vi "Check interlock status.vi"(8 "error in":errorcluster, 11 "VISA resource name":refnum<visa-resource-name>) -> (0 "error out":errorcluster, 3 "Boolean":bool)   [LabVIEW 2021]
uses:
  HI-POT_Driver/GPT-9800_GSB_L8.5/GPT-9000.lvlib
panel:
  out "Query the function test status":string
  out "Return  the test status":string
  out "RESULT":bool
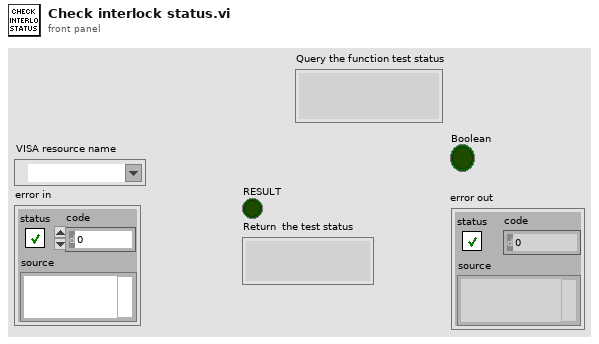
[diagram p1: front panel]
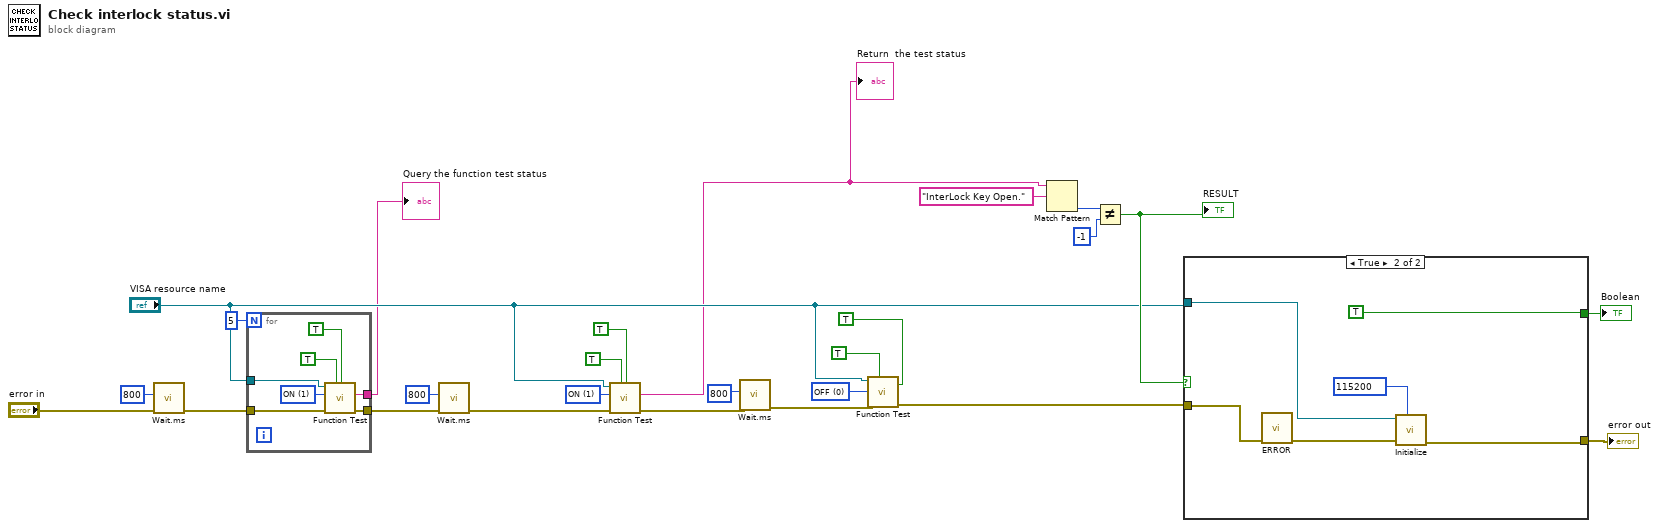
[diagram p0: block diagram]
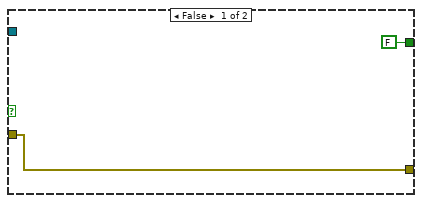
[diagram p2: hidden frame]
diagram:
  w9 = u8 1 items=["OFF", "ON"] ("Function Test")
  w18 = u8 0 items=["OFF", "ON"] ("Function Test")
  n1 = call "Wait.ms.vi"("error in"="error in", "milliseconds to wait"=u32 800) -> ("error out"=w13:errorcluster)  [unwired: 9 in]
  n2 = for {
    N: 5 -> [_]
    tunnel: "VISA resource name" -> [w28]
    tunnel: [w27] -> w2
    tunnel: w13 -> [w33]
    tunnel: [w29] -> w6
    w32 = u8 1 items=["OFF", "ON"] ("Function Test")
    n3 = call "Function Test.vi"("VISA resource name"=w28, "Function Test"=w32, "error in"=w33, "Enable to Setup"=TRUE, "Enable to Query"=TRUE) -> ("Query the function test status"=w27:string, "error out"=w29:errorcluster)  [unwired: 3 in, 1 out]
  }
  "Query the function test status" <- w2
  n4 = call "Wait.ms.vi"("error in"=w6, "milliseconds to wait"=u32 800) -> ("error out"=w8:errorcluster)  [unwired: 9 in]
  n5 = call "Function Test.vi"("VISA resource name"="VISA resource name", "Function Test"=w9, "error in"=w8, "Enable to Setup"=TRUE, "Enable to Query"=TRUE) -> ("Query the function test status"=w3:string, "error out"=w4:errorcluster)  [unwired: 3 in, 1 out]
  "Return  the test status" <- w3
  n6 = call "Wait.ms.vi"("error in"=w4, "milliseconds to wait"=u32 800) -> ("error out"=w16:errorcluster)  [unwired: 9 in]
  n7 = call "Function Test.vi"("VISA resource name"="VISA resource name", "Function Test"=w18, "error in"=w16, "Enable to Setup"=TRUE, "Enable to Query"=TRUE) -> ("error out"=w24:errorcluster)  [unwired: 3 in, 2 out]
  n8 = Match Pattern(string=w3, regular expression="InterLock Key Open.") -> (offset past match=w22:i32)  [unwired: 1 in, 3 out]
  n9 = Not Equal?(x=w22, y=-1) -> (x != y?=w17:bool)
  "RESULT" <- w17
  n10 = case shown="True" w17 {
    tunnel: [FALSE TRUE] -> w25
    tunnel: "VISA resource name" -> [_ w38]
    tunnel: [w34 w37] -> w26
    tunnel: w24 -> [w34 w36]
    frame False {
    }
    frame True {
      w40 = u32 115200 items=["9600"=9600, "19200"=19200, "38400"=38400, "57600"=57600, "115200"=115200] ("Configure RS232 Baud Rate")
      n11 = call "ERROR.vi"(8:w36) -> ("error"=w41:errorcluster)  [unwired: 10 in]
      n12 = call "Initialize.vi"("Configure RS232 Baud Rate"=w40, "error in (no error)"=w41, "VISA resource name"=w38) -> ("error out"=w37:errorcluster)  [unwired: 5 in, 3 out]
    }
  }
  "error out" <- w26
  "Boolean" <- w25
